vi "Test Assert Greater.vi"(8 "error in (no error)":errorcluster) -> (0 "error out":errorcluster)   [LabVIEW 2020]
uses:
  classes/Assert/Assert.lvclass
  classes/Test/Test.lvclass
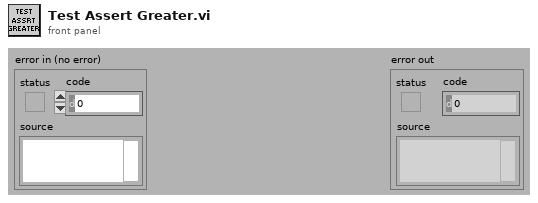
[diagram p1: front panel]
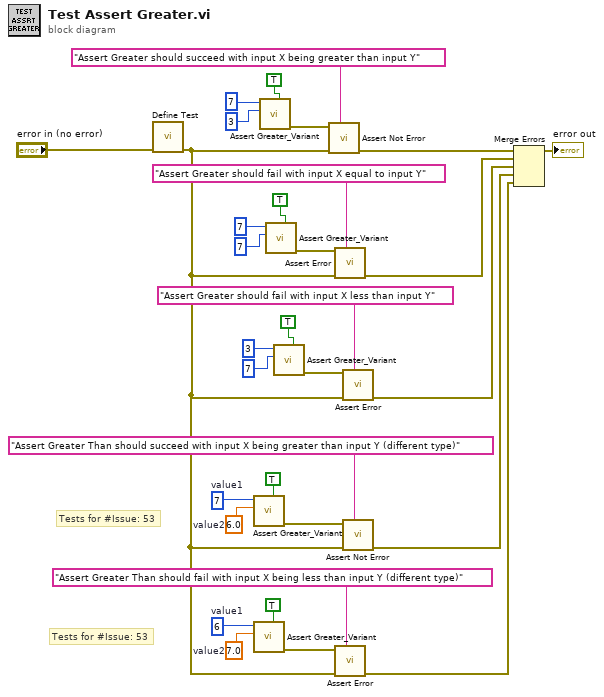
[diagram p0: block diagram]
diagram:
  w7 = 7.0  # value2
  w6 = 6  # value1
  w8 = 6.0  # value2
  w9 = 7  # value1
  # "Tests for #Issue: 53"
  # "Tests for #Issue: 53"
  n1 = call "Define Test.vi"("error in (no error)"="error in (no error)") -> ("error out"=w2:errorcluster)  [unwired: 9 in, 1 out]
  n2 = call "Assert Greater_Variant.vi"("Assert Only? (F)"=TRUE, "Y"=w8, "X"=w9) -> ("error out"=w11:errorcluster)  [unwired: 7 in, 1 out]
  n3 = call "Assert Greater_Variant.vi"("Assert Only? (F)"=TRUE, "Y"=w7, "X"=w6) -> ("error out"=w4:errorcluster)  [unwired: 7 in, 1 out]
  n4 = call "Assert Greater_Variant.vi"("Assert Only? (F)"=TRUE, "Y"=3, "X"=7) -> ("error out"=w33:errorcluster)  [unwired: 7 in, 1 out]
  n5 = call "Assert Greater_Variant.vi"("Assert Only? (F)"=TRUE, "Y"=7, "X"=7) -> ("error out"=w31:errorcluster)  [unwired: 7 in, 1 out]
  n6 = call "Assert Greater_Variant.vi"("Assert Only? (F)"=TRUE, "Y"=7, "X"=3) -> ("error out"=w20:errorcluster)  [unwired: 7 in, 1 out]
  n7 = call "Assert Not Error.vi"("Label"="Assert Greater should succeed with input X being greater than input Y", "error in (no error)"=w2, "Not Error?"=w33) -> ("error out"=w26:errorcluster)  [unwired: 7 in, 1 out]
  n8 = call "Assert Error.vi"("Label"="Assert Greater should fail with input X equal to input Y", "error in (no error)"=w2, "Error?"=w31) -> ("error out"=w15:errorcluster)  [unwired: 7 in, 1 out]
  n9 = call "Assert Error.vi"("Label"="Assert Greater Than should fail with input X being less than input Y (different type)", "error in (no error)"=w2, "Error?"=w4) -> ("error out"=w3:errorcluster)  [unwired: 7 in, 1 out]
  n10 = call "Assert Error.vi"("Label"="Assert Greater should fail with input X less than input Y", "error in (no error)"=w2, "Error?"=w20) -> ("error out"=w14:errorcluster)  [unwired: 7 in, 1 out]
  n11 = call "Assert Not Error.vi"("Label"="Assert Greater Than should succeed with input X being greater than input Y (different type)", "error in (no error)"=w2, "Not Error?"=w11) -> ("error out"=w12:errorcluster)  [unwired: 7 in, 1 out]
  n12 = Merge Errors(w26, w15, w14, w12, w3) -> (→"error out":errorcluster)
